vi "Insert SubSystem Controller.vi"(8 "error in (no error)":errorcluster, 9 "VI Refs":refnum<vi>[](array[refnum]), 10 "Project Folder":path, 11 "Application in":refnum<vi>) -> (0 "error out":errorcluster)   [LabVIEW 2023]
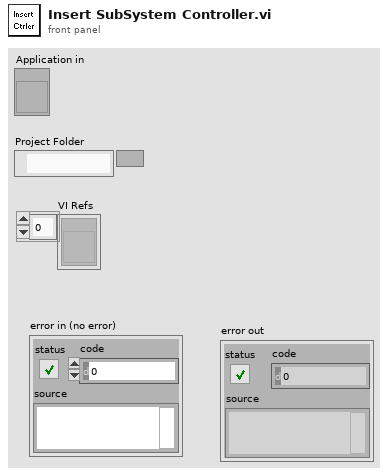
[diagram p1: front panel]
types:
  T1 = enum32{"Bad", "Idle", "Run top level", "Running"}
  T2 = cluster{"Alignment":enum32{"Left", "Right", "Hybrid", "Center", "Gravity"}, "Rules":enum32{"Strict", "Allow Wires Under Labels", "Allow Wires Under Lead Nodes", "Allow Wires Under Wide Blocks"}, "Max Heuristic Iterations":u32, "Max Simplex Iterations":u32, "Block Padding":cluster{"Horizontal":i32, "Vertical":i32}, "Wire Padding":cluster{"Horizontal":i32, "Vertical":i32}, "Auto-Tune by Topology":bool, "Fine-Tune Y Positions":bool, "Align All Controls on Left":bool, "Align All Indicators on Right":bool, "Use Array Dimension Heuristics":bool}
  T3 = typedef "LVRectTypeDef.ctl" = cluster{"Left":i16, "Top":i16, "Right":i16, "Bottom":i16}
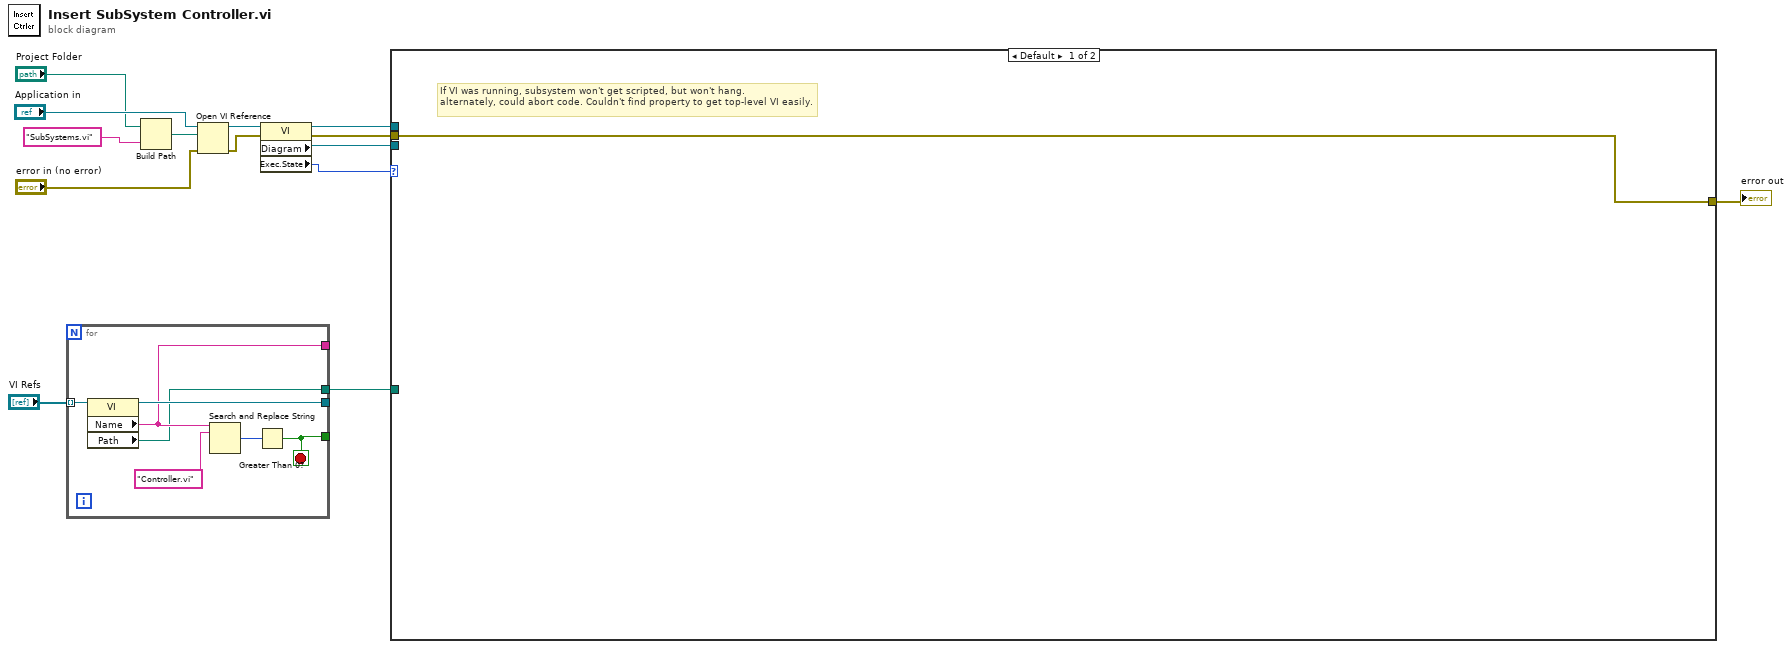
[diagram p0: block diagram]
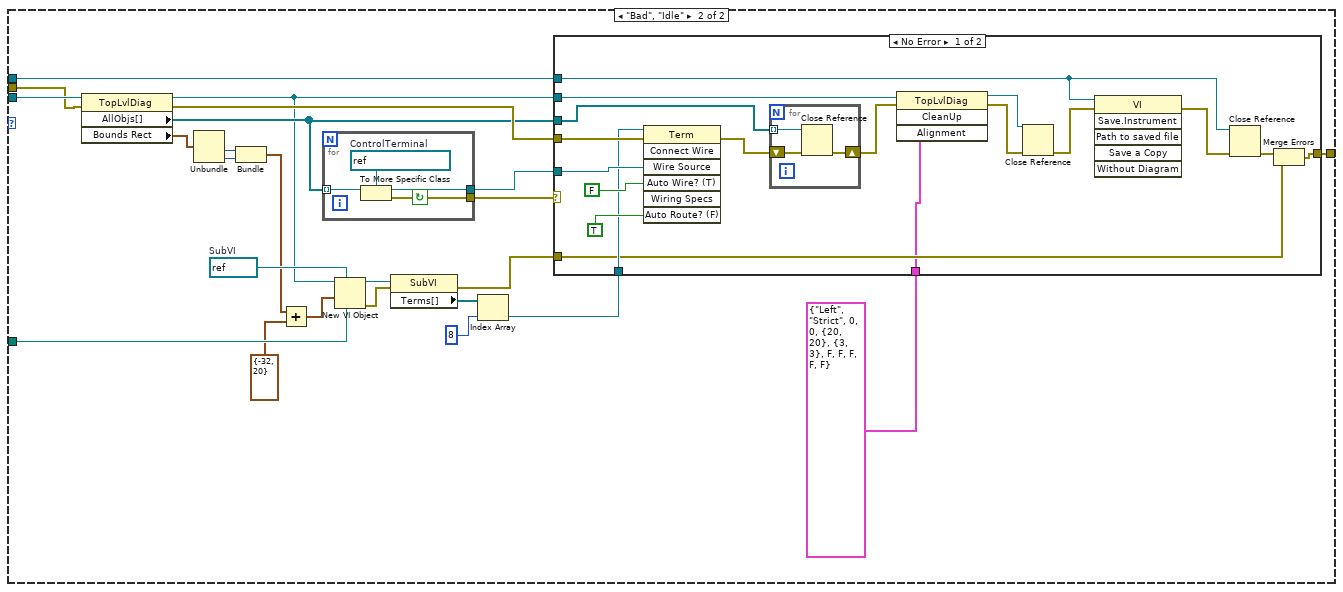
[diagram p2: hidden frame]
diagram:
  n1 = for {
    tunnel: "VI Refs" -> [w19] mode=indexing
    tunnel: [w15] -> _
    tunnel: [w18] -> _
    tunnel: [w17] -> _
    tunnel: [w16] -> w3
    stop <- w15 stop-if-true
    n2 = property class="VI"(reference=w19) -> (reference out=w18:refnum<vi>, "Name"=w17:string, "Path"=w16:path)  [unwired: 1 in, 1 out]
    n3 = Search and Replace String(input string=w17, search string="Controller.vi") -> (number of replacements=w20:i32)  [unwired: 6 in, 3 out]
    n4 = Greater Than 0?(x=w20) -> (x > 0?=w15:bool)
  }
  n5 = Build Path(base path="Project Folder", name or relative path="SubSystems.vi" ("Type")) -> (appended path=w12:path)
  n6 = Open VI Reference(application reference (local)="Application in", vi path=w12, error in (no error)="error in (no error)") -> (vi reference=w1:refnum<vi>, error out=w6:errorcluster)  [unwired: 3 in]
  n7 = property class="VI"(reference=w1, error in=w6) -> (reference out=w4:refnum<vi>, error out=w5:errorcluster, "Diagram"=w14:refnum<vi>, "Exec.State"=w2:T1)
  n8 = case shown="Default" w2 {
    tunnel: w14 -> [_ w46]
    tunnel: [w22 w45] -> w8
    tunnel: w5 -> [w22 w44]
    tunnel: w4 -> [_ w39]
    tunnel: w3 -> [_ w37]
    frame Default {
      # "If VI was running, subsystem won't get scripted, but won't hang.\nalternately, could abort code. Couldn't find property to get top-level VI easily."
    }
    frame "Bad", "Idle" {
      w38 = refnum<vi> refnum  # SubVI
      n9 = property class="TopLvlDiag"(reference=w46, error in=w44) -> (reference out=w24:refnum<vi>, error out=w43:errorcluster, "AllObjs[]"=w40:refnum<vi>[], "Bounds Rect"=w33:T3)
      n10 = Unbundle(w33) -> ("Right"=w32:i16, "Bottom"=w31:i16)  [unwired: 2 out]
      n11 = Bundle("Right"=w32, "Bottom"=w31) -> (w26:cluster{"Right":i16, "Bottom":i16})  [unwired: 1 in]
      n12 = Add(x=w26, y=cluster{"Right":i16, "Bottom":i16} {"Right"=-32, "Bottom"=20} ("output cluster")) -> (x+y=w25:cluster{"Right":i16, "Bottom":i16})
      n13 = for {
        tunnel: w40 -> [w72] mode=indexing
        tunnel: [w70] -> w41
        tunnel: [w69] -> w42
        stop <- w69 continue-if-true
        w71 = refnum<vi> refnum  # ControlTerminal
        n14 = To More Specific Class(target class=w71, reference=w72) -> (specific class reference=w70:refnum<vi>, error out=w69:errorcluster)  [unwired: 1 in]
      }
      n15 = New VI Object(vi object class=w38, owner refnum=w24, position/next to=w25, 6:w37) -> (object refnum=w36:refnum<vi>, 0:w30:errorcluster)  [unwired: 4 in]
      n16 = property class="SubVI"(reference=w36, error in=w30) -> (error out=w29:errorcluster, "Terms[]"=w35:refnum<vi>[])  [unwired: 1 out]
      n17 = Index Array(array=w35, index=8) -> (element=w34:refnum<vi>)
      n18 = case shown="No Error" w42 {
        tunnel: w24 -> [w51 _]
        tunnel: w39 -> [w54 _]
        tunnel: [w55 w68] -> w45
        tunnel: w43 -> [w63 w68]
        tunnel: w40 -> [w62 _]
        tunnel: w41 -> [w61 _]
        tunnel: w34 -> [w58 _]
        tunnel: w29 -> [w57 _]
        tunnel: T2 {"Alignment"=enum."Left", "Rules"=enum."Strict", "Max Heuristic Iterations"=0, "Max Simplex Iterations"=0, "Block Padding"={"Horizontal"=20, "Vertical"=20}, "Wire Padding"={"Horizontal"=3, "Vertical"=3}, "Auto-Tune by Topology"=FALSE, "Fine-Tune Y Positions"=FALSE, "Align All Controls on Left"=FALSE, "Align All Indicators on Right"=FALSE, "Use Array Dimension Heuristics"=FALSE} ("Clean Up Options") -> [w47 _]
        frame No Error {
          n19 = invoke class="Term" method="Connect Wire"(reference=w58, error in=w63, "Wire Source"=w61, "Auto Wire? (T)"=FALSE, "Auto Route? (F)"=TRUE) -> (error out=w64:errorcluster)  [unwired: 2 in, 6 out]
          n20 = for {
            tunnel: w62 -> [w67] mode=indexing
            shift-right: [w65] -> w48
            shift-left: w64 -> [w66]
            n21 = Close Reference(reference=w67, error in (no error)=w66) -> (error out=w65:errorcluster)
          }
          n22 = invoke class="TopLvlDiag" method="CleanUp"(reference=w51, error in=w48, "Alignment"=w47) -> (reference out=w50:refnum<vi>, error out=w49:errorcluster)  [unwired: 1 in, 2 out]
          n23 = Close Reference(reference=w50, error in (no error)=w49) -> (error out=w53:errorcluster)
          n24 = invoke class="VI" method="Save.Instrument"(reference=w54, error in=w53) -> (error out=w52:errorcluster)  [unwired: 4 in, 5 out]
          n25 = Close Reference(reference=w54, error in (no error)=w52) -> (error out=w56:errorcluster)
          n26 = Merge Errors(w56, w57) -> (w55:errorcluster)
        }
        frame Error {
        }
      }
    }
  }
  "error out" <- w8
